vi "Close VI Reference.vi"(8 "error in":errorcluster, 11 "ILabVIEWFile in":refnum<class "LabVIEW File.lvclass">) -> (0 "error out":errorcluster, 3 "ILabVIEWFile out":refnum<class "LabVIEW File.lvclass">)   [LabVIEW 2026, in "LabVIEW File.lvclass"]
doc: "Close all VI/element references of the object."
uses:
  LabVIEW File.lvclass
  LabVIEW File.lvclass/LabVIEW File.ctl
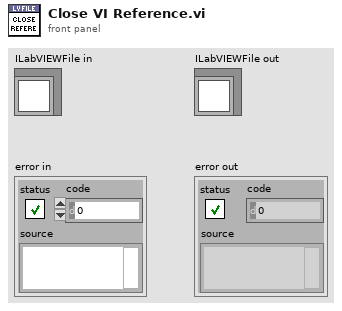
[diagram p1: front panel]
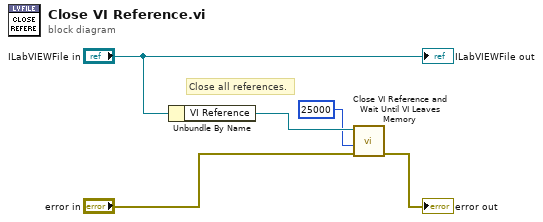
[diagram p0: block diagram]
diagram:
  # "Close all references."
  n1 = Unbundle By Name("ILabVIEWFile in") -> ("VI Reference"=w4:refnum<vi>)
  n2 = call <vilib>:"Close VI Reference and Wait Until VI Leaves Memory.vi"("error in (no error)"="error in", "Timeout (ms)"=25000, "VI reference"=w4) -> ("error out"=→"error out":errorcluster)  [unwired: 8 in]
  "ILabVIEWFile out" <- "ILabVIEWFile in"
